vi "Main.vi"() -> ()   [LabVIEW 2018]
doc: "Copyright (c) 2019, Labvolution Limited - www.labvolution.com\n\nThis software is distributed under the BSD 3-Clause License. For the full license please the LICENSE file or visit www.labvolution.com/license"
uses:
  callback-system-exec/CallbackSystemExec.vi
  callback-system-exec/callback-system-exec.lvlib
panel:
  in  "Abort command":bool
  out "Exit":bool
  in  "Execute command":bool
  out "Standard Error":string
  out "Standard Out":string
  in  "Working directory":path
  in  "Command":string
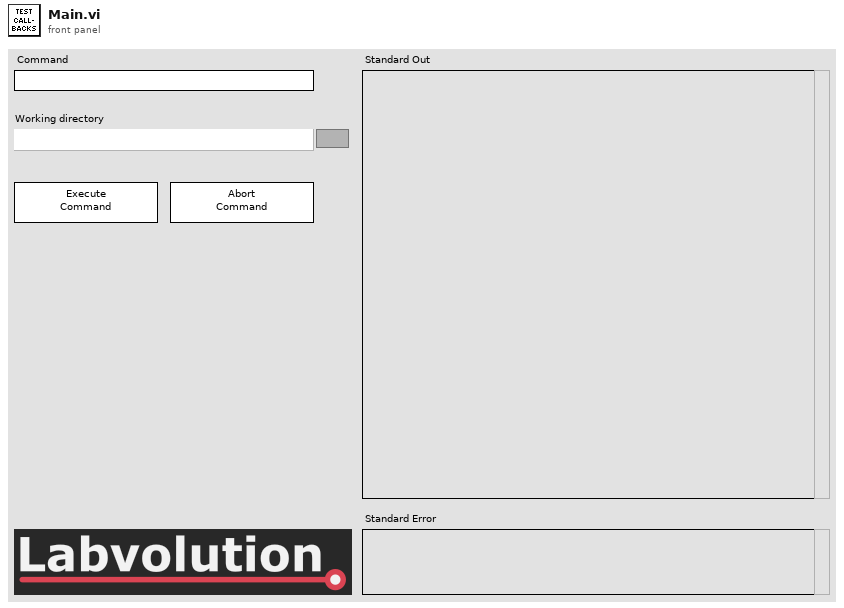
[diagram p1: front panel]
types:
  T1 = cluster{"Standard Out UE":refnum<user-event>, "Standard Error UE":refnum<user-event>, "Exited UE":refnum<user-event>}
  T2 = enum32{"invalid app kind", "Development System", "Run Time System", "Student Edition", "Embedded LabVIEW", "Evaluation", "Custom"}
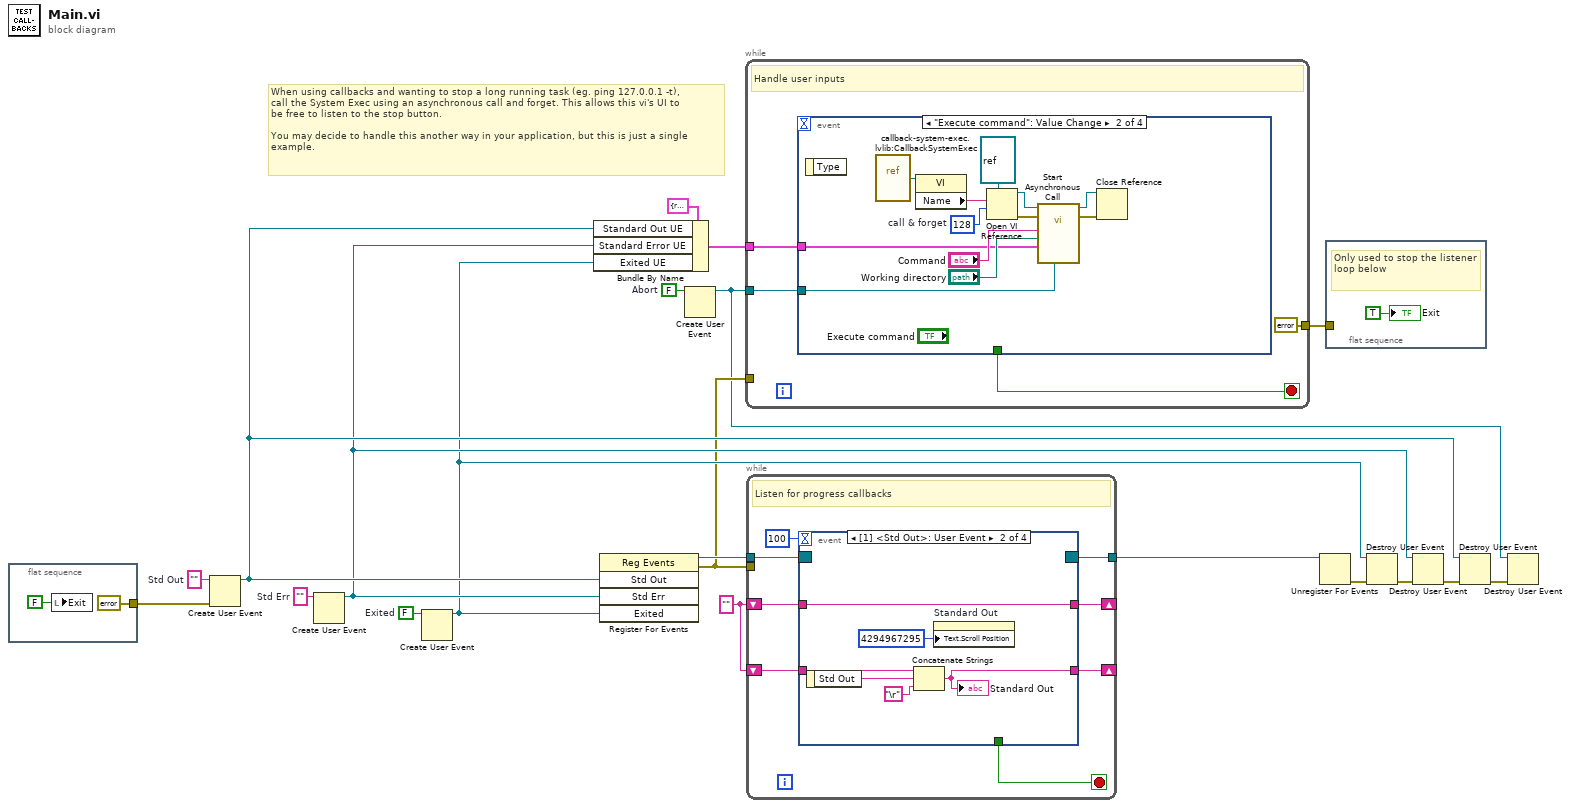
[diagram p0: block diagram]
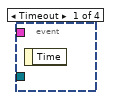
[diagram p2: hidden frame]
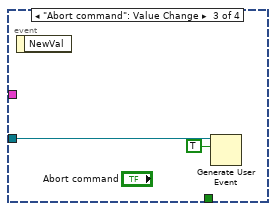
[diagram p3: hidden frame]
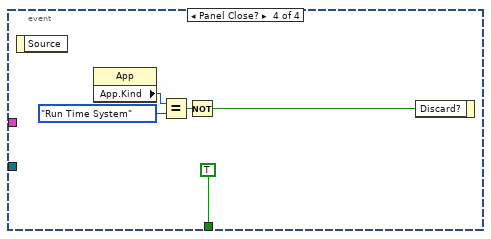
[diagram p4: hidden frame]
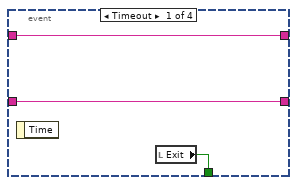
[diagram p5: hidden frame]
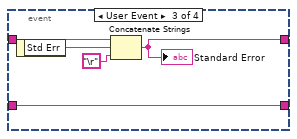
[diagram p6: hidden frame]
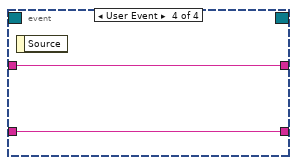
[diagram p7: hidden frame]
diagram:
  w3 = FALSE  # Abort
  w16 = ""
  w20 = FALSE  # Exited
  w19 = ""  # Std Err
  w18 = ""  # Std Out
  # "When using callbacks and wanting to stop a long running task (eg. ping 127.0.0.1 -t),\ncall the System Exec using an asynchronous call and forget. This allows this vi's UI to\nbe free to listen to the stop button.\n\nYou may decide to handle this another way in your application, but this is just a single\nexample."
  n1 = flat-sequence {
    tunnel: [errorcluster {"status"=FALSE, "code"=0, "source"=""} ("error in (no error)")] -> w7
    frame #0 {
      n2 = local write "Exit"(FALSE ("Exit")) -> ()
    }
  }
  n3 = Create User Event(user event datatype=w18, error in=w7) -> (user event=w11:refnum<user-event>)  [unwired: 1 out]
  n4 = Create User Event(user event datatype=w19) -> (user event=w10:refnum<user-event>)  [unwired: 1 in, 1 out]
  n5 = Create User Event(user event datatype=w20) -> (user event=w9:refnum<user-event>)  [unwired: 1 in, 1 out]
  n6 = Bundle By Name(cluster=T1 {"Standard Out UE"=refnum, "Standard Error UE"=refnum, "Exited UE"=refnum} ("Caller Events"), "Standard Out UE"=w11, "Standard Error UE"=w10, "Exited UE"=w9) -> (w4:T1)
  n7 = register-events(w11, w10, w9) -> (reference out=w8:refnum<event-registration>, error out=w6:errorcluster)  [unwired: 2 in]
  n8 = Create User Event(user event datatype=w3) -> (user event=w1:refnum<user-event>)  [unwired: 1 in, 1 out]
  n9 = while {
    tunnel: w4 -> [w25]
    tunnel: w6 -> [_]
    tunnel: [errorcluster {"status"=FALSE, "code"=0, "source"=""} ("error in (no error)")] -> w5
    tunnel: w1 -> [w23]
    stop <- w26 stop-if-true
    # "Handle user inputs"
    n10 = event shown="[1] \"Execute command\": Value Change" {
      selector: _ -> [_ _ _ _]
      dyn-events: _ -> [_ _ _ _]
      timeout: _ -> [_ _ _ _]
      tunnel: [_ _ _ TRUE] -> w26
      tunnel: w25 -> [_ w30 _ _]
      tunnel: w23 -> [_ w29 w40 _]
      event Timeout {
        n11 = event-data() -> ()  [unwired: 1 in, 1 out]
      }
      event "Execute command": Value Change {
        w34 = 128  # call & forget
        n12 = event-data() -> ()  [unwired: 1 in, 1 out]
        n13 = vi-ref "callback-system-exec.lvlib:CallbackSystemExec.vi"() -> (w36:refnum<vi>)
        n14 = property class="VI"(reference=w36) -> ("Name"=w35:string)  [unwired: 1 in, 2 out]
        n15 = Open VI Reference(type specifier VI Refnum (for type only)=refnum<vi> refnum, vi path=w35, options=w34) -> (vi reference=w37:refnum<vi>, error out=w38:errorcluster)  [unwired: 3 in]
        n16 = call-by-ref "Start Asynchronous Call"(reference=w37, error in=w38, "Abort UE"=w29, "Caller Events"=w30, "Working directory"="Working directory", "Command"="Command") -> (reference out=w27:refnum<vi>, error out=w28:errorcluster)  [unwired: 5 in, 3 out]
        n17 = Close Reference(reference=w27, error in (no error)=w28) -> ()  [unwired: 1 out]
      }
      event "Abort command": Value Change {
        n18 = event-data() -> ()  [unwired: 1 in, 1 out]
        n19 = Generate User Event(user event=w40, event data cluster=TRUE ("event data")) -> ()  [unwired: 2 in, 2 out]
      }
      event Panel Close? {
        n20 = event-data() -> ()  [unwired: 1 in, 1 out]
        n21 = property class="App"() -> ("App.Kind"=w44:T2)  [unwired: 2 in, 2 out]
        n22 = Equal?(x=w44, y=T2."Run Time System") -> (x = y?=w42:bool)
        n23 = Not(x=w42) -> (.not. x?=w41:bool)
        n24 = event-data("Discard?"=w41) -> ()  [unwired: 1 in, 1 out]
      }
    }
  }
  n25 = while {
    tunnel: [w52] -> w12
    shift-right: [w50] -> _
    shift-left: w16 -> [w51]
    shift-right: [w49] -> _
    shift-left: w16 -> [w48]
    tunnel: w8 -> [w47]
    tunnel: w6 -> [_]
    stop <- w53 stop-if-true
    # "Listen for progress callbacks"
    n26 = event shown="[1] <Std Out>: User Event" {
      selector: w47 -> [_ _ _ _]
      dyn-events: [_ _ _ _] -> w52
      timeout: 100 -> [_ _ _ _]
      tunnel: [w54 _ _ _] -> w53
      tunnel: w51 -> [w55 w61 w67 w69]
      tunnel: [w55 w58 w67 w69] -> w50
      tunnel: [w56 w59 w63 w68] -> w49
      tunnel: w48 -> [w56 w59 w65 w68]
      event Timeout {
        n27 = event-data() -> ()  [unwired: 1 in, 1 out]
        n28 = local read "Exit"() -> (w54:bool)
      }
      event User Event {
        n29 = event-data() -> ("Std Out"=w60:string)  [unwired: 1 in]
        n30 = Concatenate Strings(w61, w60, "\r") -> (w58:string)
        "Standard Out" <- w58
        n31 = property on="Standard Out" class="Str"("Text.Scroll Position"=u32 4294967295) -> ()  [unwired: 2 in, 2 out]
      }
      event User Event {
        n32 = event-data() -> ("Std Err"=w64:string)  [unwired: 1 in]
        n33 = Concatenate Strings(w65, w64, "\r") -> (w63:string)
        "Standard Error" <- w63
      }
      event User Event {
        n34 = event-data() -> ()  [unwired: 1 in, 1 out]
      }
    }
  }
  n35 = Unregister For Events(event registration refnum=w12) -> (error out=w13:errorcluster)  [unwired: 1 in]
  n36 = flat-sequence {
    tunnel: w5 -> [_]
    frame #0 {
      # "Only used to stop the listener loop below"
      "Exit" <- TRUE ("Exit")
    }
  }
  n37 = Destroy User Event(user event=w9, error in=w13) -> (error out=w14:errorcluster)
  n38 = Destroy User Event(user event=w10, error in=w14) -> (error out=w15:errorcluster)
  n39 = Destroy User Event(user event=w11, error in=w15) -> (error out=w2:errorcluster)
  n40 = Destroy User Event(user event=w1, error in=w2) -> ()  [unwired: 1 out]
